vi "RemoteVI Fixture Arrange.vi"(0 "Fixture":path, 5 "Tab Panel":path, 11 "error in":errorcluster) -> (15 "error out":errorcluster)   [LabVIEW 2020]
doc: "Build tool of RemoteVI Fixture.vi: run it ONCE after composing the fixture (aixml\\compose_fixture.py), with the fixture idle. AIXML cannot create a tab control, so this copies the tab control of Tab Panel (a VI whose panel holds only a tab control labelled Tab with empty pages One and Two - see aixml\\RemoteVI Fixture Prep Tab Panel.xml) onto the fixture's panel, then lays the panel out: the controls in a column on the left (Switch, Button, Number, Text, Mode, Stop, then Ask and Open below Stop; empty space right of Stop), Graph and Tab to their right, List right of Tab, no overlap, and error out at the bottom right, ending 4 px inside the 900 x 600 window (Panel Bounds), which LabVIEW gives a scroll range of about 6 px both ways (it scrolls 10 px past the last object, measured), so both scrollbars can scroll the panel - by so little that every click of the tests still hits its control when the panel was scrolled (the mouse wheel over Number scrolls the panel too, as it does locally); Number without increment/decrement buttons, Text limited to one line, Graph with its palette visible, List (a single-column multicolumn listbox) with the rows Alpha, Beta, Gamma, Delta, four rows high, no column headers, no horizontal scrollbar, label visible (Bounds is read-only on it, error 1029), Button with the tip strip Press me, tabs of a fixed 80 px width (Tab Size 2 = fixed, measured), Switch switch when pressed, Button, Ask, Open and Stop latch when released, fixed-width tabs; window origin 0,0. Saves the fixture."
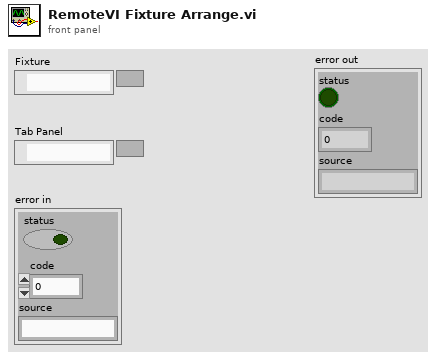
[diagram p1: front panel]
types:
  T1 = cluster{"Left":i32, "Top":i32, "Right":i32, "Bottom":i32}
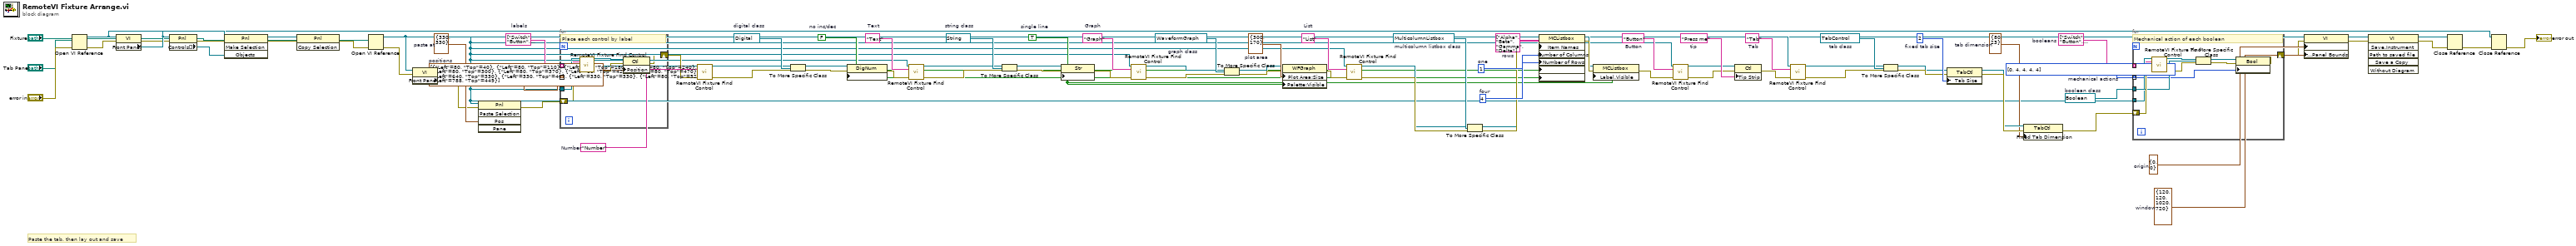
[diagram p0: block diagram]
diagram:
  w79 = T1 {"Left"=120, "Top"=120, "Right"=1020, "Bottom"=720}  # window
  w78 = cluster{"Horizontal":i32, "Vertical":i32} {"Horizontal"=0, "Vertical"=0}  # origin
  w76 = refnum<vi> refnum  # boolean class
  w75 = i32[] [0, 4, 4, 4, 4]  # mechanical actions
  w74 = string[] ["Switch", "Button", "Ask", "Open", "Stop"]  # booleans
  w70 = cluster{"Width":i32, "Height":i32} {"Width"=80, "Height"=23}  # tab dimension
  w69 = 2  # fixed tab size
  w66 = refnum<vi> refnum  # tab class
  w63 = "Tab"  # Tab
  w61 = "Press me"  # tip
  w58 = "Button"  # Button
  w54 = 4  # four
  w53 = 1  # one
  w52 = string[][] [["Alpha"], ["Beta"], ["Gamma"], ["Delta"]]  # rows
  w49 = refnum<vi> refnum  # multicolumn listbox class
  w46 = "List"  # List
  w44 = cluster{"Width":i32, "Height":i32} {"Width"=300, "Height"=170}  # plot area
  w41 = refnum<vi> refnum  # graph class
  w38 = "Graph"  # Graph
  w36 = TRUE  # single line
  w33 = refnum<vi> refnum  # string class
  w30 = "Text"  # Text
  w28 = FALSE  # no inc/dec
  w25 = refnum<vi> refnum  # digital class
  w22 = "Number"  # Number
  w20 = cluster{"Left":i32, "Top":i32}[] [{"Left"=80, "Top"=40}, {"Left"=80, "Top"=110}, {"Left"=80, "Top"=180}, {"Left"=80, "Top"=240}, {"Left"=80, "Top"=300}, {"Left"=80, "Top"=370}, {"Left"=80, "Top"=420}, {"Left"=80, "Top"=470}, {"Left"=640, "Top"=330}, {"Left"=330, "Top"=40}, {"Left"=330, "Top"=330}, {"Left"=80, "Top"=520}, {"Left"=788, "Top"=449}]  # positions
  w19 = string[] ["Switch", "Button", "Number", "Text", "Mode", "Stop", "Ask", "Open", "List", "Graph", "Tab", "Log Path", "error out"]  # labels
  w17 = cluster{"Left":i32, "Top":i32} {"Left"=330, "Top"=330}  # paste at
  # "Paste the tab, then lay out and save"
  n1 = Open VI Reference(vi path="Tab Panel", error in (no error)="error in") -> (vi reference=w4:refnum<vi>, error out=w5:errorcluster)  [unwired: 4 in]
  n2 = property class="VI"(reference=w4, error in=w5) -> (error out=w6:errorcluster, "Front Panel"=w7:refnum<vi>)  [unwired: 1 out]
  n3 = property class="Pnl"(reference=w7, error in=w6) -> (error out=w8:errorcluster, "Controls[]"=w9:refnum<vi>[])  [unwired: 1 out]
  n4 = invoke class="Pnl" method="Make Selection"(reference=w7, error in=w8, "Objects"=w9) -> (reference out=w10:refnum<vi>, error out=w11:errorcluster)  [unwired: 1 in, 2 out]
  n5 = invoke class="Pnl" method="Copy Selection"(reference=w10, error in=w11) -> (error out=w12:errorcluster)  [unwired: 1 in, 2 out]
  n6 = Open VI Reference(vi path="Fixture", error in (no error)=w12) -> (vi reference=w13:refnum<vi>, error out=w14:errorcluster)  [unwired: 4 in]
  n7 = property class="VI"(reference=w13, error in=w14) -> (error out=w15:errorcluster, "Front Panel"=w16:refnum<vi>)  [unwired: 1 out]
  n8 = invoke class="Pnl" method="Paste Selection"(reference=w16, error in=w15, "Pos"=w17) -> (error out=w18:errorcluster)  [unwired: 2 in, 4 out]
  n9 = for {
    tunnel: w19 -> [w86] mode=indexing
    tunnel: w20 -> [w87] mode=indexing
    tunnel: w16 -> [w88]
    shift-right: [w90] -> w21
    shift-left: w18 -> [w89]
    # "Place each control by label"
    n10 = call "RemoteVI Fixture Find Control.vi"("Panel"=w88, "label"=w86, "error in"=w89) -> ("Control Ref"=w91:refnum<vi>, "error out"=w92:errorcluster)  [unwired: 11 in]
    n11 = property class="Ctl"(reference=w91, error in=w92, "Position"=w87) -> (error out=w90:errorcluster)  [unwired: 1 out]
  }
  n12 = call "RemoteVI Fixture Find Control.vi"("Panel"=w16, "label"=w22, "error in"=w21) -> ("Control Ref"=w23:refnum<vi>, "error out"=w24:errorcluster)  [unwired: 11 in]
  n13 = To More Specific Class(target class=w25, reference=w23, error in=w24) -> (specific class reference=w26:refnum<vi>, error out=w27:errorcluster)
  n14 = property class="DigNum"(reference=w26, error in=w27, "Increment/Decrement Visible?"=w28) -> (error out=w29:errorcluster)  [unwired: 1 out]
  n15 = call "RemoteVI Fixture Find Control.vi"("Panel"=w16, "label"=w30, "error in"=w29) -> ("Control Ref"=w31:refnum<vi>, "error out"=w32:errorcluster)  [unwired: 11 in]
  n16 = To More Specific Class(target class=w33, reference=w31, error in=w32) -> (specific class reference=w34:refnum<vi>, error out=w35:errorcluster)
  n17 = property class="Str"(reference=w34, error in=w35, "Limit To Single Line?"=w36) -> (error out=w37:errorcluster)  [unwired: 1 out]
  n18 = call "RemoteVI Fixture Find Control.vi"("Panel"=w16, "label"=w38, "error in"=w37) -> ("Control Ref"=w39:refnum<vi>, "error out"=w40:errorcluster)  [unwired: 11 in]
  n19 = To More Specific Class(target class=w41, reference=w39, error in=w40) -> (specific class reference=w42:refnum<vi>, error out=w43:errorcluster)
  n20 = property class="WFGraph"(reference=w42, error in=w43, "Plot Area:Size"=w44, "Palette:Visible"=w36) -> (error out=w45:errorcluster)  [unwired: 1 out]
  n21 = call "RemoteVI Fixture Find Control.vi"("Panel"=w16, "label"=w46, "error in"=w45) -> ("Control Ref"=w47:refnum<vi>, "error out"=w48:errorcluster)  [unwired: 11 in]
  n22 = To More Specific Class(target class=w49, reference=w47, error in=w48) -> (specific class reference=w50:refnum<vi>, error out=w51:errorcluster)
  n23 = property class="MCListbox"(reference=w50, error in=w51, "Item Names"=w52, "Number of Columns"=w53, "Number of Rows"=w54, "Visible Items:Column Headers Visible"=w28, "Visible Items:Horizontal Scrollbar Visible"=w28) -> (reference out=w55:refnum<vi>, error out=w56:errorcluster)
  n24 = property class="MCListbox"(reference=w55, error in=w56, "Label.Visible"=w36) -> (error out=w57:errorcluster)  [unwired: 1 out]
  n25 = call "RemoteVI Fixture Find Control.vi"("Panel"=w16, "label"=w58, "error in"=w57) -> ("Control Ref"=w59:refnum<vi>, "error out"=w60:errorcluster)  [unwired: 11 in]
  n26 = property class="Ctl"(reference=w59, error in=w60, "Tip Strip"=w61) -> (error out=w62:errorcluster)  [unwired: 1 out]
  n27 = call "RemoteVI Fixture Find Control.vi"("Panel"=w16, "label"=w63, "error in"=w62) -> ("Control Ref"=w64:refnum<vi>, "error out"=w65:errorcluster)  [unwired: 11 in]
  n28 = To More Specific Class(target class=w66, reference=w64, error in=w65) -> (specific class reference=w67:refnum<vi>, error out=w68:errorcluster)
  n29 = property class="TabCtl"(reference=w67, error in=w68, "Tab Size"=w69) -> (reference out=w71:refnum<vi>, error out=w72:errorcluster)
  n30 = property class="TabCtl"(reference=w71, error in=w72, "Fixed Tab Dimension"=w70) -> (error out=w73:errorcluster)  [unwired: 1 out]
  n31 = for {
    tunnel: w74 -> [w93] mode=indexing
    tunnel: w75 -> [w94] mode=indexing
    tunnel: w76 -> [w96]
    tunnel: w16 -> [w95]
    shift-right: [w98] -> w77
    shift-left: w73 -> [w97]
    # "Mechanical action of each boolean"
    n32 = call "RemoteVI Fixture Find Control.vi"("Panel"=w95, "label"=w93, "error in"=w97) -> ("Control Ref"=w99:refnum<vi>, "error out"=w100:errorcluster)  [unwired: 11 in]
    n33 = To More Specific Class(target class=w96, reference=w99, error in=w100) -> (specific class reference=w101:refnum<vi>, error out=w102:errorcluster)
    n34 = property class="Bool"(reference=w101, error in=w102, "Mechanical Action"=w94) -> (error out=w98:errorcluster)  [unwired: 1 out]
  }
  n35 = property class="VI"(reference=w13, error in=w77, "Front Panel Window:Origin"=w78, "Front Panel Window:Panel Bounds"=w79) -> (reference out=w80:refnum<vi>, error out=w81:errorcluster)
  n36 = invoke class="VI" method="Save.Instrument"(reference=w80, error in=w81) -> (reference out=w82:refnum<vi>, error out=w83:errorcluster)  [unwired: 4 in, 4 out]
  n37 = Close Reference(reference=w82, error in (no error)=w83) -> (error out=w84:errorcluster)
  n38 = Close Reference(reference=w4, error in (no error)=w84) -> (error out=→"error out":errorcluster)
